vi "Consumer.vi"(8 "error in (no error)":errorcluster, 9 "Data":variant, 10 "Case ID":string, 11 "uService Template in":refnum<class "TCP Listener.lvclass">) -> (0 "error out":errorcluster, 3 "uService Template out":refnum<class "TCP Listener.lvclass">)   [LabVIEW 2020, in "TALOS.lvlib" / "TCP Listener.lvlib" / "TCP Listener.lvclass"]
uses:
  TCP Listener.lvclass
  TCP Listener Consumer Case Selector.ctl
  TALOS.lvlib
  C:/Users/marco/Documents/GitHub_Lab/TALOS/talos/Father of all uServices/Father of all uServices/Father of all uServices.lvclass
  Father of all uServices/Father of all uServices/Father of all uServices.lvclass
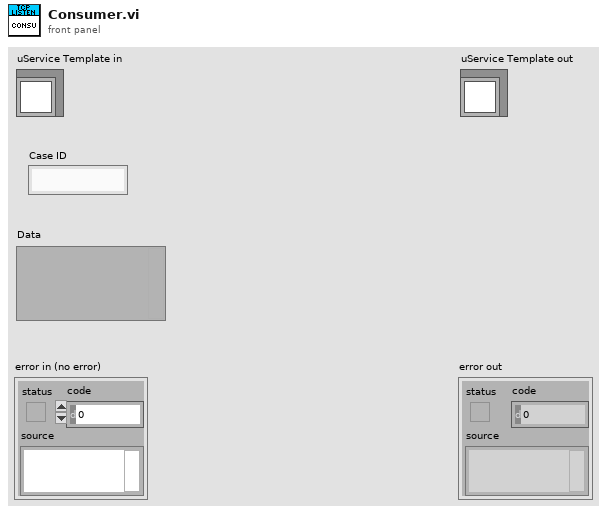
[diagram p1: front panel]
types:
  T1 = typedef "TALOS.lvlib/TCP Listener.lvlib/TCP Listener.lvclass/TCP Listener Consumer Case Selector.ctl" = enum16{"Set Client ID", "Listen", "Idle"}
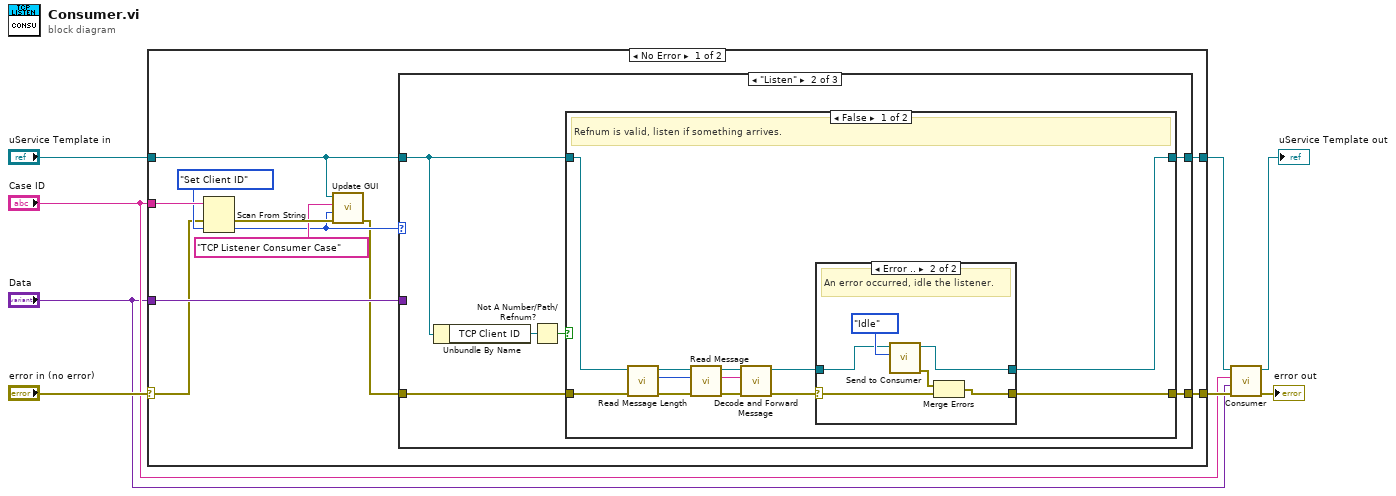
[diagram p0: block diagram]
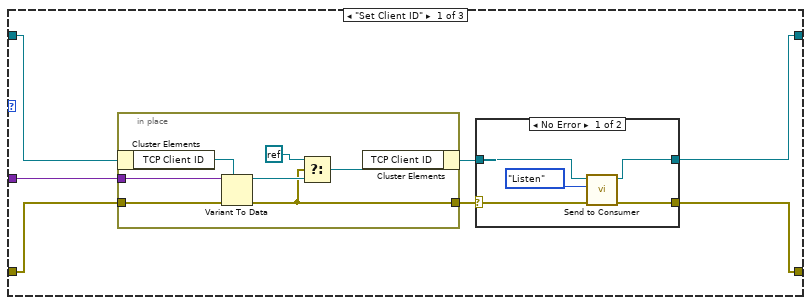
[diagram p2: hidden frame]
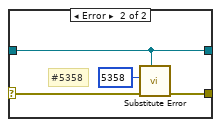
[diagram p3: hidden frame]
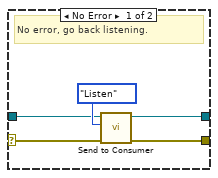
[diagram p4: hidden frame]
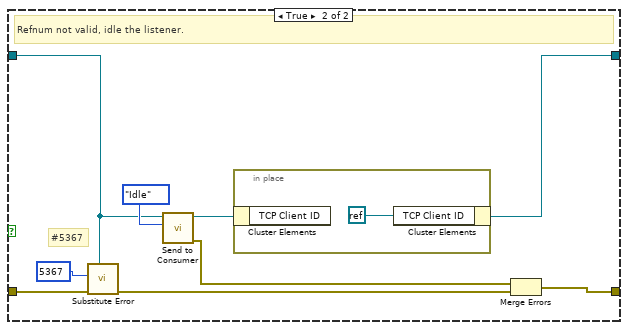
[diagram p5: hidden frame]
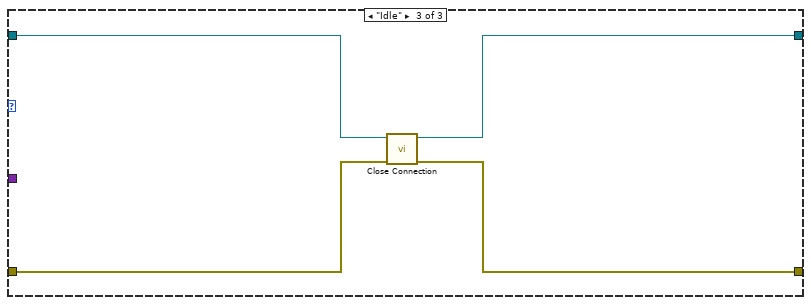
[diagram p6: hidden frame]
diagram:
  n1 = case shown="No Error" "error in (no error)" {
    selector: "error in (no error)" -> [w10 w86]
    tunnel: "uService Template in" -> [w14 w87]
    tunnel: [w17 w87] -> w4
    tunnel: [w18 w86] -> w3
    tunnel: "Case ID" -> [w16 _]
    tunnel: "Data" -> [w19 _]
    frame No Error {
      n2 = Scan From String(input string=w16, error in=w10, default 1=TCP_Listener_Consumer_Case_Selector."Set Client ID") -> (error out=w13:errorcluster, output 1=w11:T1)  [unwired: 2 in, 2 out]
      n3 = call "Update GUI.vi"("error in (no error)"=w13, "Data"=w11, "GUI Item Name"="TCP Listener Consumer Case", "uService Template in"=w14) -> ("error out"=w9:errorcluster)  [unwired: 6 in, 1 out]
      n4 = case shown="\"Listen\"" w11 {
        tunnel: w19 -> [w26 _ _]
        tunnel: w14 -> [w25 w47 w85]
        tunnel: [w23 w48 w83] -> w18
        tunnel: [w21 w46 w84] -> w17
        tunnel: w9 -> [w20 w43 w82]
        frame "Set Client ID" {
          n5 = in-place "In Place Element Structure" {
            in-place-border: w26 -> [w42]
            in-place-border: w20 -> [w41]
            in-place-border: [w37] -> w24
            n6 = in-place-cluster #1(w25) -> ("TCP Client ID"=w38:refnum<k5>)
            n7 = Variant To Data(error in=w41, type=w38, Variant=w42) -> (data=w40:refnum<k5>, error out=w37:errorcluster)
            n8 = Select(t=refnum<k0> refnum, s=w37, f=w40) -> (s? t:f=w39:refnum<k5>)
            n9 = in-place-cluster #1("TCP Client ID"=w39) -> (w22:refnum<class "TCP Listener.lvclass">)
          }
          n10 = case shown="No Error" w24 {
            selector: w24 -> [w30 w34]
            tunnel: [w29 w33] -> w23
            tunnel: w22 -> [w28 w32]
            tunnel: [w27 w32] -> w21
            frame No Error {
              n11 = call "Send to Consumer.vi"("error in (no error)"=w30, "Case ID"=TCP_Listener_Consumer_Case_Selector."Listen" ("TCP Listener Consumer Case Selector"), "uService Template in"=w28) -> ("error out"=w29:errorcluster, "uService Template out"=w27:refnum<class "TCP Listener.lvclass">)  [unwired: 7 in]
            }
            frame Error {
              # "#5358"
              n12 = call "Substitute Error.vi"("LabVIEW Object"=w32, "error in (no error)"=w34, "Error Code"=5358) -> ("error out"=w33:errorcluster)  [unwired: 8 in]
            }
          }
        }
        frame "Listen" {
          n13 = Unbundle By Name(w47) -> ("TCP Client ID"=w45:refnum<k5>)
          n14 = Not A Number/Path/Refnum?(number/path/refnum=w45) -> (NaN/Path/Refnum?=w44:bool)
          n15 = case shown="False" w44 {
            tunnel: w43 -> [w60 w76]
            tunnel: [w53 w78] -> w48
            tunnel: w47 -> [w59 w75]
            tunnel: [w50 w72] -> w46
            frame False {
              # "Refnum is valid, listen if something arrives."
              n16 = call-dynamic "Read Message Length.vi"("error in (no error)"=w60, "TCP Listener in"=w59) -> ("error out"=w57:errorcluster, "Bytes to read"=w56:i32, "TCP Listener out"=w58:refnum<class "TCP Listener.lvclass">)  [unwired: 7 in]
              n17 = call-dynamic "Read Message.vi"("error in (no error)"=w57, "Bytes to read"=w56, "TCP Listener in"=w58) -> ("error out"=w51:errorcluster, "Message string"=w49:string, "TCP Listener out"=w52:refnum<class "TCP Listener.lvclass">)  [unwired: 6 in]
              n18 = call-dynamic "Decode and Forward Message.vi"("error in (no error)"=w51, "Message undecoded"=w49, "TCP Listener in"=w52) -> ("error out"=w55:errorcluster, "TCP Listener out"=w54:refnum<class "TCP Listener.lvclass">)  [unwired: 7 in]
              n19 = case shown="Error .." w55 {
                selector: w55 -> [w64 w68]
                tunnel: w54 -> [w63 w70]
                tunnel: [w62 w67] -> w53
                tunnel: [w61 w66] -> w50
                frame No Error {
                  # "No error, go back listening."
                  n20 = call "Send to Consumer.vi"("error in (no error)"=w64, "Case ID"=TCP_Listener_Consumer_Case_Selector."Listen" ("TCP Listener Consumer Case Selector"), "uService Template in"=w63) -> ("error out"=w62:errorcluster, "uService Template out"=w61:refnum<class "TCP Listener.lvclass">)  [unwired: 7 in]
                }
                frame Error {
                  # "An error occurred, idle the listener."
                  n21 = call "Send to Consumer.vi"("Case ID"=TCP_Listener_Consumer_Case_Selector."Idle" ("TCP Listener Consumer Case Selector"), "uService Template in"=w70) -> ("error out"=w69:errorcluster, "uService Template out"=w66:refnum<class "TCP Listener.lvclass">)  [unwired: 8 in]
                  n22 = Merge Errors(w69, w68) -> (w67:errorcluster)
                }
              }
            }
            frame True {
              # "#5367"
              # "Refnum not valid, idle the listener."
              n23 = call "Substitute Error.vi"("LabVIEW Object"=w75, "error in (no error)"=w76, "Error Code"=5367) -> ("error out"=w77:errorcluster)  [unwired: 8 in]
              n24 = call "Send to Consumer.vi"("Case ID"=TCP_Listener_Consumer_Case_Selector."Idle" ("TCP Listener Consumer Case Selector"), "uService Template in"=w75) -> ("error out"=w79:errorcluster, "uService Template out"=w73:refnum<class "TCP Listener.lvclass">)  [unwired: 8 in]
              n25 = in-place {
                n26 = in-place-cluster #2(w73) -> ()  [unwired: 1 out]
                n27 = in-place-cluster #2("TCP Client ID"=refnum<k0> refnum) -> (w72:refnum<class "TCP Listener.lvclass">)
              }
              n28 = Merge Errors(w79, w77) -> (w78:errorcluster)
            }
          }
        }
        frame "Idle" {
          n29 = call-dynamic "Close Connection.vi"("error in"=w82, "uService Template in"=w85) -> ("error out"=w83:errorcluster, "uService Template out"=w84:refnum<class "TCP Listener.lvclass">)  [unwired: 8 in]
        }
      }
    }
    frame Error {
    }
  }
  n30 = call-parent "Consumer.vi"("error in (no error)"=w3, "Data"="Data", "Case ID"="Case ID", "uService Template in"=w4) -> ("error out"=→"error out":errorcluster, "uService Template out"=→"uService Template out":refnum<class "TCP Listener.lvclass">)  [unwired: 6 in]
